vi "Update caption.vi"(7 "Interpret as Unicode (T)":bool=TRUE, 8 "error in (no error)":errorcluster, 10 "Caption In":string, 11 "Control Reference In":refnum<vi>) -> (1 "error out":errorcluster, 3 "Control Reference Out":refnum<vi>)   [LabVIEW 2019, in "Language Selection.lvlib"]
doc: "Uses \"Caption In\" input string to translate the caption of the control wired as input.\n- - -\nCopyright (c) 2026, Merecs Engineering GmbH"
uses:
  Language Selection.lvlib
panel:
  # "Connector Pane"
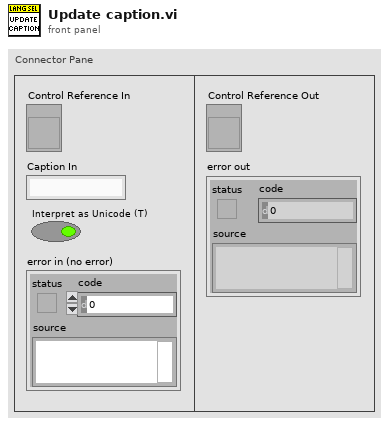
[diagram p1: front panel]
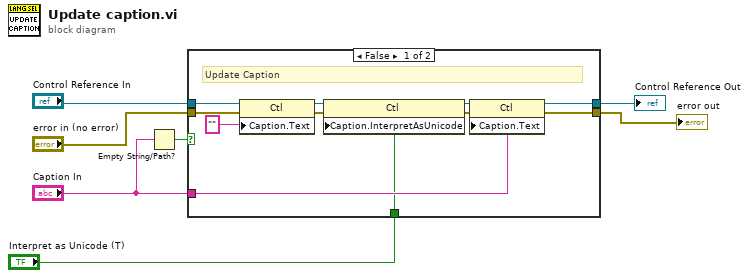
[diagram p0: block diagram]
diagram:
  n1 = Empty String/Path?(string/path="Caption In") -> (empty?=w6:bool)
  n2 = case shown="False" w6 {
    tunnel: "Control Reference In" -> [w16 w20]
    tunnel: "error in (no error)" -> [w13 w19]
    tunnel: "Caption In" -> [w12 _]
    tunnel: [w18 w20] -> w1
    tunnel: [w17 w19] -> w2
    tunnel: "Interpret as Unicode (T)" -> [w10 _]
    frame False {
      # "Update Caption"
      n3 = property class="Ctl"(reference=w16, error in=w13, "Caption.Text"="") -> (reference out=w15:refnum<vi>, error out=w14:errorcluster)
      n4 = property class="Ctl"(reference=w15, error in=w14, "Caption.InterpretAsUnicode"=w10) -> (reference out=w9:refnum<vi>, error out=w8:errorcluster)
      n5 = property class="Ctl"(reference=w9, error in=w8, "Caption.Text"=w12) -> (reference out=w18:refnum<vi>, error out=w17:errorcluster)
    }
    frame True {
    }
  }
  "error out" <- w2
  "Control Reference Out" <- w1
